vi "Main_RT_V2.vi"() -> ()   [LabVIEW 2018]
uses:
  enum_Main_RT_V2.ctl
  <vilib>/Platform/TimedLoop/XDataNode/timing_clust.ctl
  <vilib>/Platform/TimedLoop/XDataNode/nitl_modes.ctl
  <vilib>/Platform/TimedLoop/XDataNode/wakeup.ctl
  enum_bras.ctl
  <vilib>/myRIO/Instrument Drivers/Onboard IO/DIO/typedefs/DIO Reference.ctl
  <vilib>/myRIO/Common/Instrument Driver Framework/Utilities/typedefs/myRIO Generic Hardware Reference.ctl
  <vilib>/myRIO/Common/Instrument Driver Framework/Utilities/typedefs/Hardware Version Enum.ctl
  <vilib>/myRIO/Common/Instrument Driver Framework/Utilities/typedefs/myRIO v1.0 Reference.ctl
  <vilib>/myRIO/Common/Instrument Driver Framework/Utilities/typedefs/Generic FPGA Reference.ctl
  <vilib>/myRIO/Common/Instrument Driver Framework/myRIO v1.0/DIO/typedefs/DIO Channels List.ctl
  <vilib>/myRIO/Common/Instrument Driver Framework/myRIO v1.0/DIO/typedefs/DIO Channels Enum.ctl
  <vilib>/userdefined/High Color/nirio_resource_hc.ctl
  enum_RT_Virage.ctl
  enum_RT_Seaux.ctl
  enum_RT_recule.ctl
  enum_RT_trieur_Balles.ctl
  enum_RT_lanceur.ctl
  <vilib>/myRIO/Common/Instrument Driver Framework/Utilities/vis/Is FPGA Ref Available.vi
  <vilib>/myRIO/Common/Instrument Driver Framework/myRIO v1.0/DIO/vis/myRIO v1.1 Open DIO.vi
  <vilib>/myRIO/Instrument Drivers/Onboard IO/DIO/vis/Read.vi
  <vilib>/myRIO/Common/Instrument Driver Framework/Utilities/vis/Validate Channels.vi
  <vilib>/myRIO/Common/Instrument Driver Framework/myRIO v1.0/DIO/vis/myRIO v1.0 Reserve DIO.vi
  <vilib>/myRIO/Common/Instrument Driver Framework/myRIO v1.0/Resource Manager/vis/myRIO v1.0 Reserve Channel List.vi
  <vilib>/myRIO/Common/Instrument Driver Framework/myRIO v1.0/DIO/vis/myRIO v1.0 Build MUX Configuration DIO.vi
  <vilib>/myRIO/Common/Instrument Driver Framework/myRIO v1.0/Resource Manager/vis/myRIO v1.0 Reserve Channel.vi
  <vilib>/myRIO/Common/Instrument Driver Framework/myRIO v1.0/Resource Manager/vis/myRIO v1.0 Unreserve Channel.vi
  <vilib>/myRIO/Common/Instrument Driver Framework/myRIO v1.0/Resource Manager/vis/myRIO v1.0 Create Configuration List.vi
  <vilib>/myRIO/Common/Instrument Driver Framework/myRIO v1.0/Resource Manager/vis/myRIO v1.0 Build Mutex Name.vi
  <vilib>/Utility/VariantDataType/GetNumericInfo.vi
  <vilib>/Utility/error.llb/Error Cluster From Error Code.vi
  <vilib>/myRIO/Common/Instrument Driver Framework/myRIO v1.0/myRIO v1.1 Open.vi
  <vilib>/myRIO/Common/Instrument Driver Framework/Utilities/vis/IO Manager.vi
  <vilib>/myRIO/Common/Instrument Driver Framework/Utilities/vis/Configuration Manager.vi
  <vilib>/myRIO/Common/Instrument Driver Framework/myRIO v1.0/Resource Manager/vis/myRIO v1.0 Configure IO.vi
  <vilib>/myRIO/Common/Instrument Driver Framework/myRIO v1.0/myRIO v1.0 Close.vi
  <vilib>/myRIO/Common/Instrument Driver Framework/myRIO v1.0/DIO/vis/myRIO v1.0 Read DIO.vi
  <vilib>/Platform/TimedLoop/XDataNode/XDataNode.xnode
  <vilib>/myRIO/Express VI/Onboard Devices/Button/Button Express VI.xnode
  <vilib>/myRIO/Instrument Drivers/Onboard IO/DIO/vis/myRIO DIO Open.xnode
  <vilib>/Platform/TimedLoop/XDataNode/XDNodeRunTimeDep.lvlib
  <vilib>/myRIO/Instrument Drivers/Onboard IO/DIO/DIO.lvlib
panel:
  in  "stop":bool
  out "Sceaux":bool
  out "Lanceur de balles":bool
  out "Virage 4":bool
  out "Virage 3":bool
  out "Clapets 2":bool
  out "Trieur de Balles":bool
  out "Reculer":bool
  out "Virage 2":bool
  out "Virage 1":bool
  out "Clapets 1":bool
  out "Detection suiveur de ligne":bool[](array[boolean])
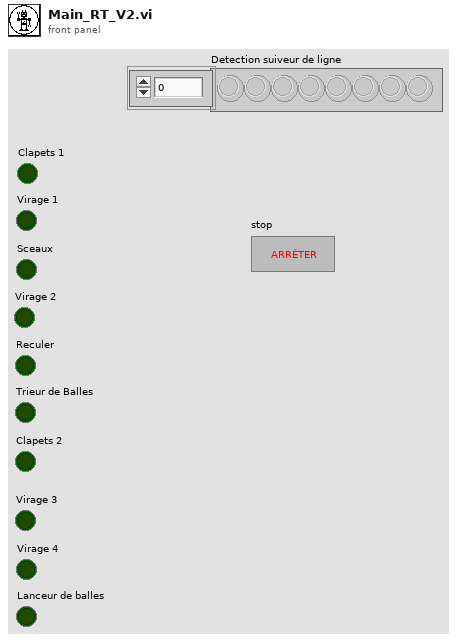
[diagram p1: front panel]
types:
  T1 = typedef "enum_Main_RT_V2.ctl" = enum16{"Initialisation", "Clapet 1", "Virage 1", "Seaux", "Virage 2", "Reculer", "Trieur Balles", "Avancer", "Clapet 2", "Virage 3", "Avancer 2", "Virage 4", "Lancer de Balles", "Arret du robot"}
  T2 = typedef "XDNodeRunTimeDep.lvlib/timing_clust.ctl" = cluster{"Expected End [f-1]":u64, "Actual End [f-1]":u64, "Finished Late? [f-1]":bool, "Expected End [i-1]":u64, "Actual End [i-1]":u64, "Finished Late? [i-1]":bool, "Expected Start [i]":u64, "Actual Start [i]":u64, "Expected Start [f]":u64, "Actual Start [f]":u64, "Source Name":string, "Structure Name":string, "Period":i64, "Deadline":i64, "Offset":i64, "Start":i64, "Priority":i32, "Timeout":i32, "Mode":T3, "Wakeup Reason":T4, "Error":errorcluster, "Source Type":string, "Secondary Source Type":string, "Global End Time":u64, "Global Start Time":u64, "Frame Duration":u64, "Iteration Duration":u64, "Assigned CPU":i32, "I/O Scan Engine Mode":u32}
  T3 = typedef "XDNodeRunTimeDep.lvlib/nitl_modes.ctl" = enum32{"No Change", "Process missed periods, maintain original phase", "Discard missed periods, maintain original phase", "Process missed periods, ignore original phase", "Discard missed periods, ignore original phase"}
  T4 = typedef "XDNodeRunTimeDep.lvlib/wakeup.ctl" = enum32{"Normal", "Aborted", "Asynchronous wakeup", "Timing source error", "Timed loop error", "Timeout"}
  T5 = typedef "enum_bras.ctl" = enum16{"Depart Bras", "Clapet Bras", "Inactif Bras", "Seaux Bras"}
  T6 = typedef "DIO.lvlib/DIO Reference.ctl" = cluster{"myRIO Reference":T7, "DIO Channels List":T11}
  T7 = typedef "myRIO Generic Hardware Reference.ctl" = cluster{"myRIO Model":T8, "myRIO Hardware Reference":T9}
  T8 = typedef "Hardware Version Enum.ctl" = enum16{"Unknown", "myRIO-1900", "myRIO-1950", "roboRIO", "NI ELVIS RIO CM", "ELVIS III"}
  T9 = typedef "myRIO v1.0 Reference.ctl" = cluster{"Generic FPGA Reference":T10, "Allow multiple opens":bool}
  T10 = typedef "Generic FPGA Reference.ctl" = refnum<k20>
  T11 = typedef "DIO Channels List.ctl" = T12[]
  T12 = typedef "DIO Channels Enum.ctl" = enum16{"Not Connected", "C/DIO0", "C/DIO1", "C/DIO2", "C/DIO3", "C/DIO4", "C/DIO5", "C/DIO6", "C/DIO7", "A/DIO0", "A/DIO1", "A/DIO2", "A/DIO3", "A/DIO4", "A/DIO5", "A/DIO6", "A/DIO7", "A/DIO8", "A/DIO9", "A/DIO10", "A/DIO11", "A/DIO12", "A/DIO13", "A/DIO14", "A/DIO15", "A/DIO16", "A/DIO17", "A/DIO18", "A/DIO19", "B/DIO0", "B/DIO1", "B/DIO2", "B/DIO3", "B/DIO4", "B/DIO5", "B/DIO6", "B/DIO7", "B/DIO8", "B/DIO9", "B/DIO10", "B/DIO11", "B/DIO12", "B/DIO13", "B/DIO14", "B/DIO15", "B/DIO16", "B/DIO17", "B/DIO18", "B/DIO19", "LED0", "LED1", "LED2", "LED3", "Button0", "DIO/DIO0", "DIO/DIO1", "DIO/DIO2", "DIO/DIO3", "DIO/DIO4", "DIO/DIO5", "DIO/DIO6", "DIO/DIO7", "DIO/DIO8", "DIO/DIO9", "SPI/CS0", "SPI/CS1", "SPI/CS2", "SPI/CS3", "LED RADIO (Green)", "LED RADIO (Red)", "LED COMM (Green)", "LED COMM (Red)", "LED MODE (Green)", "LED MODE (Red)"}
  T13 = typedef "nirio_resource_hc.ctl" = tag
  T14 = typedef "enum_RT_Virage.ctl" = enum16{"Avancer", "STOP", "Lacher Ligne", "Tourner"}
  T15 = typedef "enum_RT_Seaux.ctl" = enum16{"Avancé 1", "Ready to Start", "Stop moteur", "Bras Inactif 1", "Frappe sceau", "Bras Inactif 2", "Avancé 2"}
  T16 = typedef "enum_RT_recule.ctl" = enum16{"Avancer", "Reculer", "STOP"}
  T17 = typedef "enum_RT_trieur_Balles.ctl" = enum16{"Initialisation", "Couleur", "Rotation1", "Rotation2", "Ouverture", "Fermeture"}
  T18 = typedef "enum_RT_lanceur.ctl" = enum16{"eloignement", "arret_robot", "moteur_lanceur", "distributeur", "arret_distributeur_lanceur"}
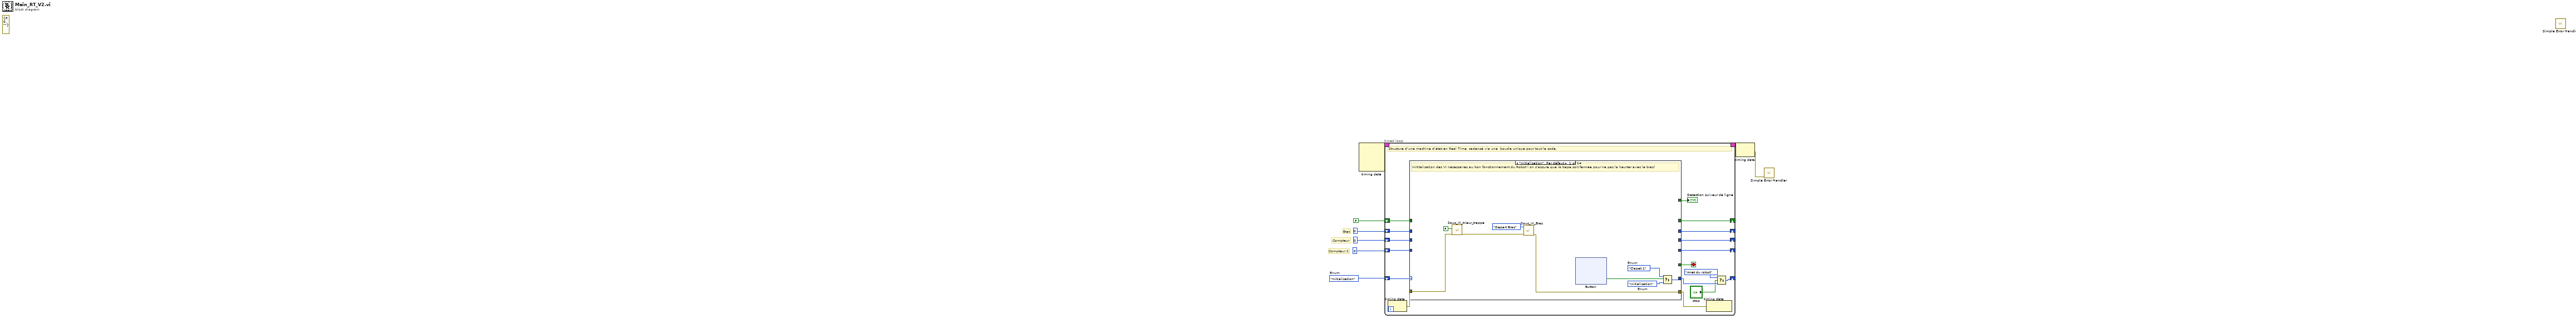
[diagram p0: block diagram]
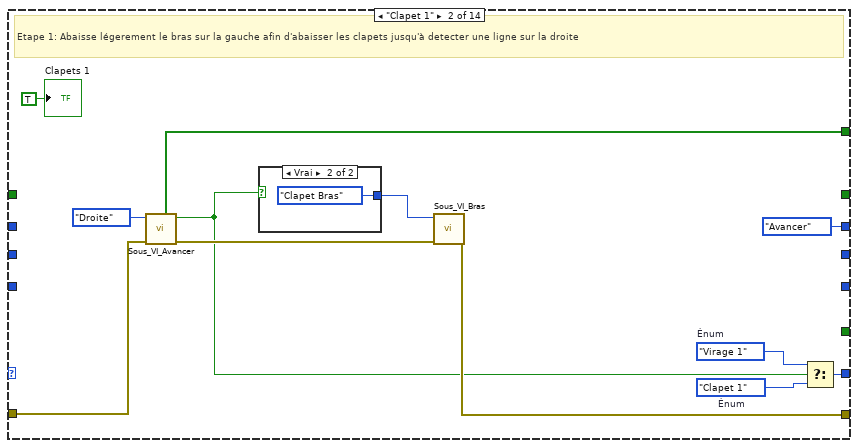
[diagram p2: hidden frame]
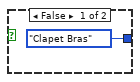
[diagram p3: hidden frame]
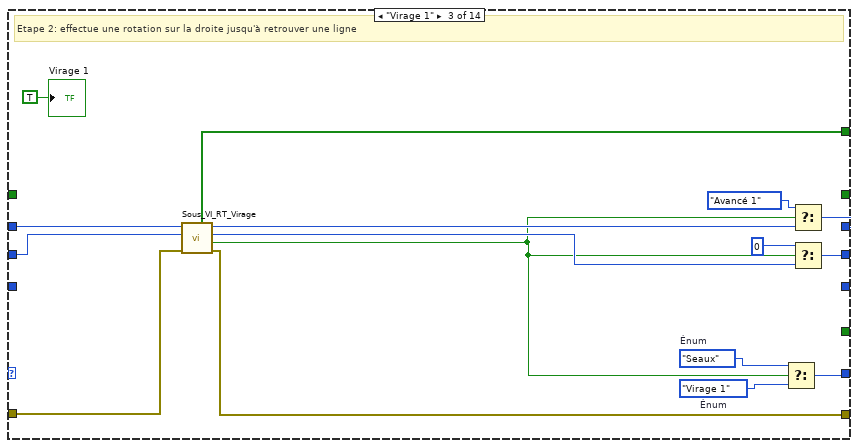
[diagram p4: hidden frame]
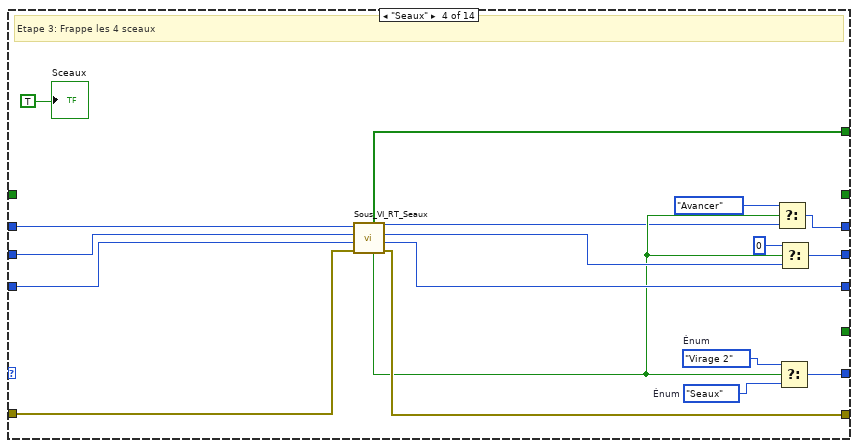
[diagram p5: hidden frame]
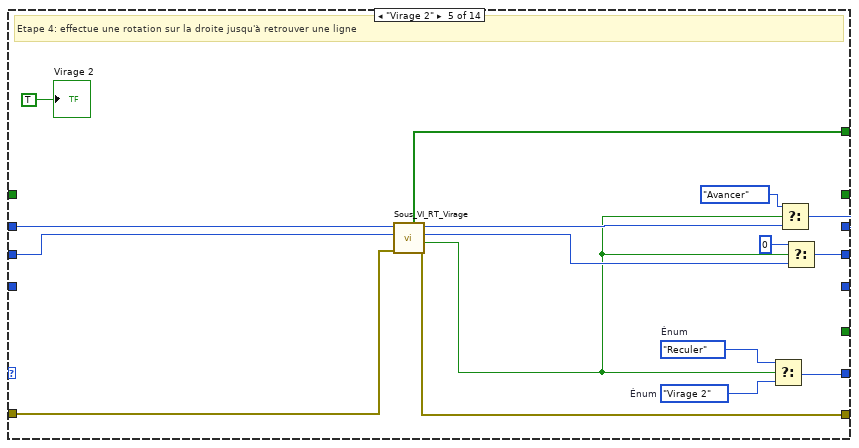
[diagram p6: hidden frame]
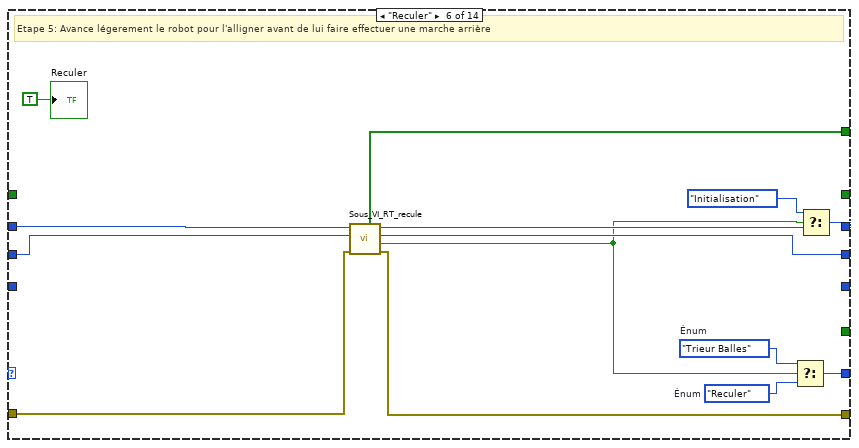
[diagram p7: hidden frame]
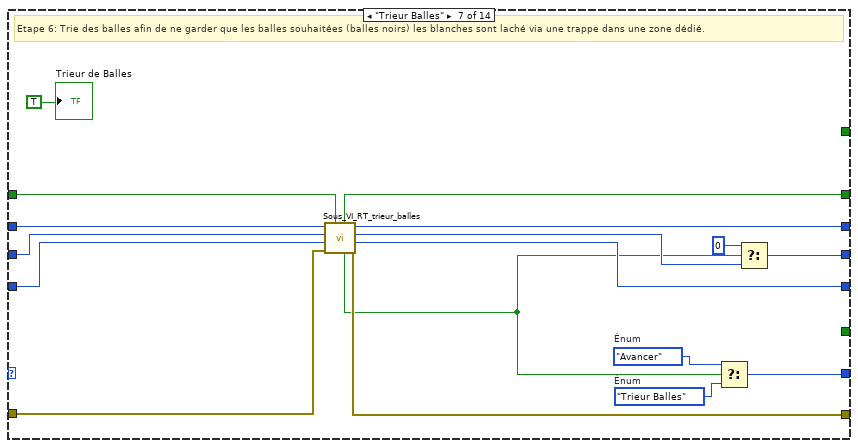
[diagram p8: hidden frame]
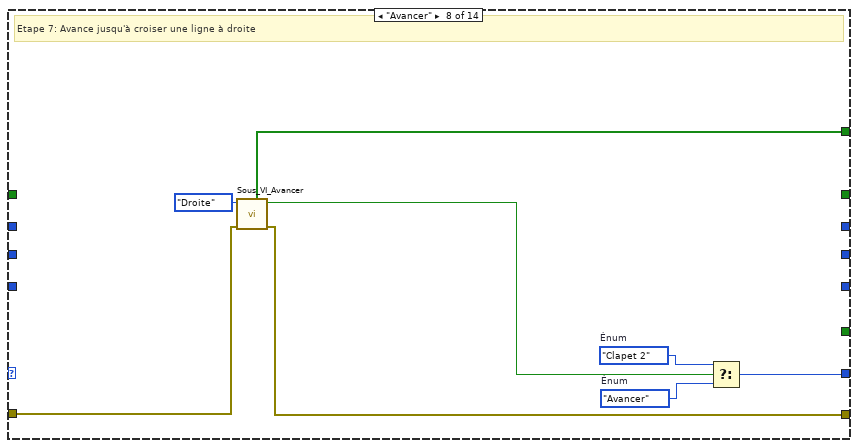
[diagram p9: hidden frame]
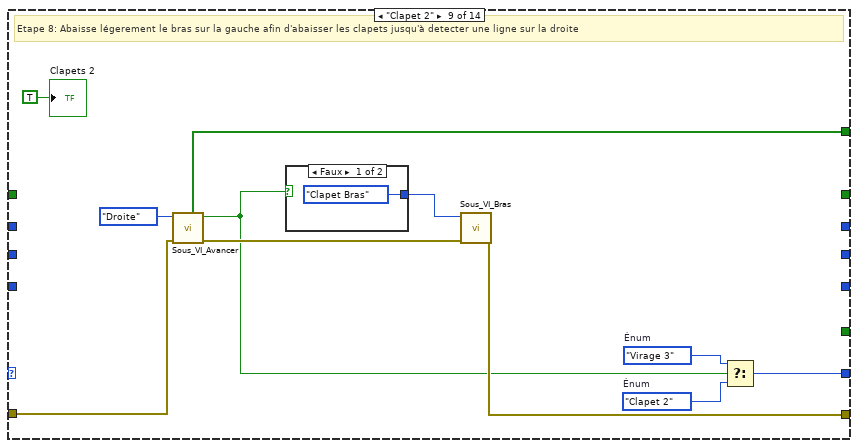
[diagram p10: hidden frame]
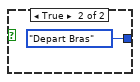
[diagram p11: hidden frame]
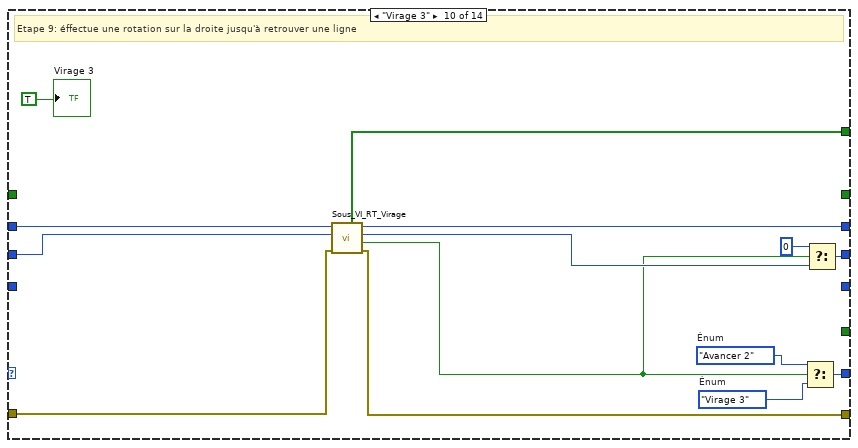
[diagram p12: hidden frame]
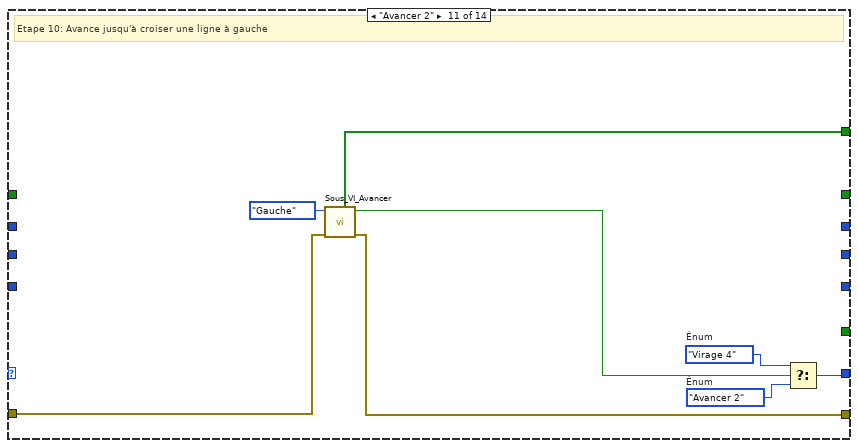
[diagram p13: hidden frame]
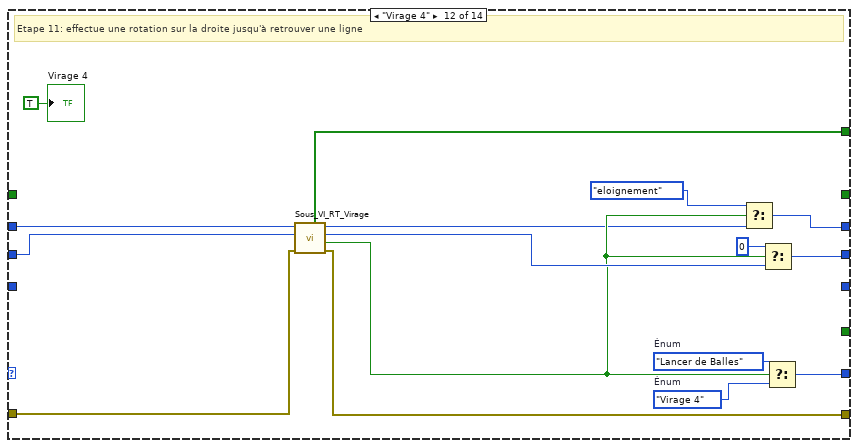
[diagram p14: hidden frame]
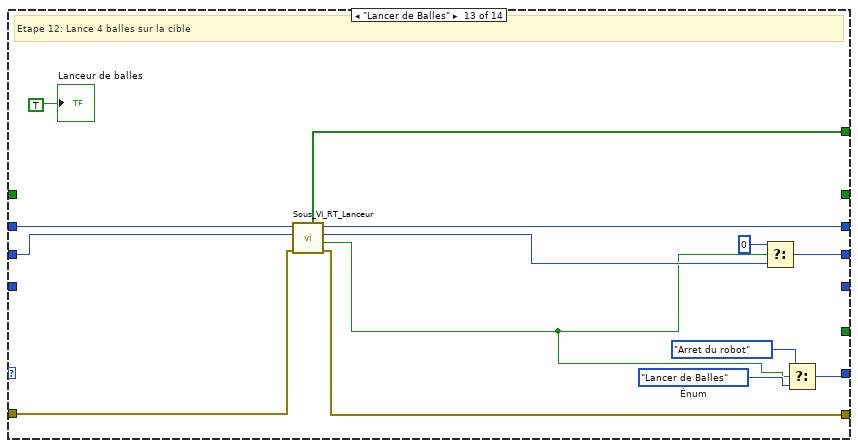
[diagram p15: hidden frame]
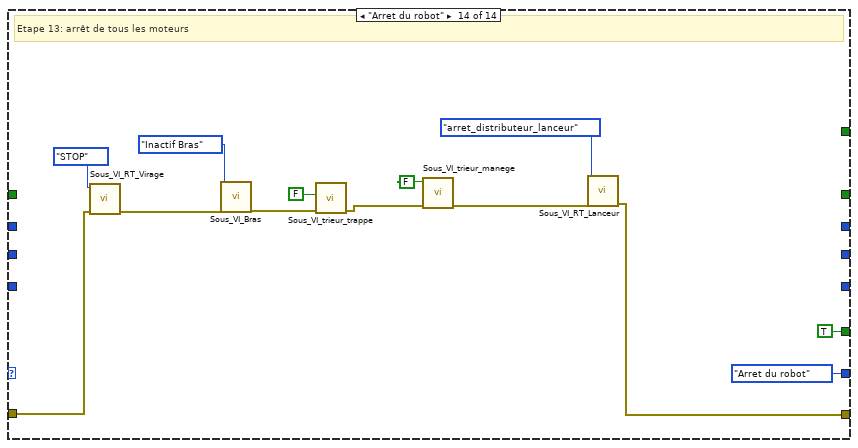
[diagram p16: hidden frame]
diagram:
  w1 = enum_Main_RT_V2."Initialisation"  # Énum
  (unwired) errorcluster {"status"=FALSE, "code"=0, "source"=""} ("error in (no error)")
  # "Compteur 2"
  # "Compteur"
  # "Etat"
  n1 = node-c288() -> (w8:T2)  [unwired: 4 in]
  n2 = timed-loop "Boucle cadencée" {
    timing: w8 -> [_]
    timing-out: [_] -> w7
    shift-right: [w22] -> _
    shift-left: u16 0 ("Etat OUT") -> [w20]
    shift-right: [w21] -> _
    shift-left: 0 -> [w19]
    shift-right: [w17] -> _
    shift-left: 0 -> [w18]
    shift-right: [w15] -> _
    shift-left: FALSE -> [w16]
    shift-right: [w12] -> _
    shift-left: w1 -> [w25]
    stop <- w14 stop-if-true
    # "Structure d'une machine d'état en Real Time, cadencé via une  boucle unique pour tout le code."
    n3 = node-c288() -> (w24:errorcluster)  [unwired: 1 in]
    n4 = case "Structure Condition" shown="\"Initialisation\", Par défaut" w25 {
      tunnel: w24 -> [w31 w78 w99 w117 w133 w144 w157 w171 w180 w196 w206 w221 w234 w250]
      tunnel: [w30 w77 w98 w116 w132 w143 w156 w170 w179 w195 w205 w220 w233 w240] -> w23
      tunnel: [_ enum_RT_Virage."Avancer" ("Etat IN") w90 w103 w121 w137 w163 _ _ w197 _ w211 w236 _] -> w22
      tunnel: [_ _ w96 w112 w128 w145 w154 _ _ w193 _ w218 w231 _] -> w21
      tunnel: w20 -> [_ _ w92 w108 w131 w147 w164 _ _ w199 _ w223 w237 _]
      tunnel: w19 -> [_ _ w97 w115 w130 w146 w162 _ _ w198 _ w222 w235 _]
      tunnel: w18 -> [_ _ _ w114 _ _ w161 _ _ _ _ _ _ _]
      tunnel: [_ _ _ w113 _ _ w160 _ _ _ _ _ _ _] -> w17
      tunnel: w16 -> [_ _ _ _ _ _ w159 _ _ _ _ _ _ _]
      tunnel: [_ _ _ _ _ _ w158 _ _ _ _ _ _ _] -> w15
      tunnel: [_ _ _ _ _ _ _ _ _ _ _ _ _ TRUE ("vi_fini")] -> w14
      tunnel: [w29 w73 w87 w107 w124 w141 w150 w169 w178 w189 w204 w215 w227 enum_Main_RT_V2."Arret du robot" ("Énum")] -> w11
      tunnel: [_ w75 w93 w109 w126 w142 _ w167 w176 w190 w202 w216 w229 _] -> w13
      frame "Initialisation", Default {
        w27 = enum_Main_RT_V2."Clapet 1"  # Énum
        w28 = enum_Main_RT_V2."Initialisation"  # Énum
        # "Inititalisation des VI nécessaires au bon fonctionnement du Robot ( on s'assure que la trape soit fermée pour ne pas la heurter avec le bras)"
        n5 = call "Sous_VI_trieur_trappe.vi"("error in (no error)"=w31, "Ouvrir"=FALSE) -> ("error out"=w32:errorcluster)  [unwired: 9 in]
        n6 = call "Sous_VI_Bras.vi"("error in (no error)"=w32, "Enum bras"=enum_bras."Depart Bras") -> ("error out"=w30:errorcluster)  [unwired: 9 in]
        n7 = xnode "Button"() -> ("Value"=w26:bool)  [unwired: 1 in, 1 out]
        n8 = Select(t=w27, s=w26, f=w28) -> (s? t:f=w29:T1)
      }
      frame "Clapet 1" {
        w71 = enum_Main_RT_V2."Clapet 1"  # Énum
        w70 = enum_Main_RT_V2."Virage 1"  # Énum
        # "Etape 1: Abaisse légerement le bras sur la gauche afin d'abaisser les clapets jusqu'à detecter une ligne sur la droite"
        n9 = call "Sous_VI_Avancer.vi"("error in (no error)"=w78, "Énum"=enum16{"Droite", "Gauche"}."Droite") -> ("error out"=w79:errorcluster, "Info de fin de Parcours"=w76:bool, "Détection ligne"=w75:bool[])  [unwired: 7 in]
        n10 = case shown="Vrai" w76 {
          tunnel: [enum_bras."Clapet Bras" ("Enum bras") enum_bras."Clapet Bras" ("Enum bras")] -> w80
          frame False {
          }
          frame True {
          }
        }
        n11 = call "Sous_VI_Bras.vi"("error in (no error)"=w79, "Enum bras"=w80) -> ("error out"=w77:errorcluster)  [unwired: 9 in]
        n12 = Select(t=w70, s=w76, f=w71) -> (s? t:f=w73:T1)
        "Clapets 1" <- TRUE
      }
      frame "Virage 1" {
        w85 = enum_Main_RT_V2."Virage 1"  # Énum
        w84 = enum_Main_RT_V2."Seaux"  # Énum
        # "Etape 2: effectue une rotation sur la droite jusqu'à retrouver une ligne"
        n13 = call "Sous_VI_RT_Virage.vi"("Erreur in"=w99, "Compteur IN"=w97, "Etat IN"=w92) -> ("Erreur out"=w98:errorcluster, "Information de fin de process"=w89:bool, "Compteur OUT"=w94:i32, "Etat OUT"=w91:T14, "Detection suiveur de ligne"=w93:bool[])  [unwired: 4 in]
        n14 = Select(t=w84, s=w89, f=w85) -> (s? t:f=w87:T1)
        n15 = Select(t=enum_RT_Seaux."Avancé 1" ("Etat IN"), s=w89, f=w91) -> (s? t:f=w90:u16)
        n16 = Select(t=0, s=w89, f=w94) -> (s? t:f=w96:i32)
        "Virage 1" <- TRUE
      }
      frame "Seaux" {
        w104 = enum_Main_RT_V2."Seaux"  # Énum
        w105 = enum_Main_RT_V2."Virage 2"  # Énum
        # "Etape 3: Frappe les 4 sceaux"
        n17 = call "Sous_VI_RT_Seaux.vi"("Erreur IN"=w117, "Nombre Sceau IN"=w114, "Compteur IN"=w115, "Etat IN"=w108) -> ("Erreur OUT"=w116:errorcluster, "Nombre Sceau OUT"=w113:i32, "Compteur OUT"=w110:i32, "Etat OUT"=w100:T15, "Indicateur de fin de process"=w102:bool, "Détection ligne"=w109:bool[])  [unwired: 2 in]
        n18 = Select(t=enum_RT_Virage."Avancer" ("Etat IN"), s=w102, f=w100) -> (s? t:f=w103:u16)
        n19 = Select(t=w105, s=w102, f=w104) -> (s? t:f=w107:T1)
        n20 = Select(t=0, s=w102, f=w110) -> (s? t:f=w112:i32)
        "Sceaux" <- TRUE
      }
      frame "Virage 2" {
        w122 = enum_Main_RT_V2."Reculer"  # Énum
        w123 = enum_Main_RT_V2."Virage 2"  # Énum
        # "Etape 4: effectue une rotation sur la droite jusqu'à retrouver une ligne"
        n21 = call "Sous_VI_RT_Virage.vi"("Erreur in"=w133, "Compteur IN"=w130, "Etat IN"=w131) -> ("Erreur out"=w132:errorcluster, "Information de fin de process"=w119:bool, "Compteur OUT"=w127:i32, "Etat OUT"=w120:T14, "Detection suiveur de ligne"=w126:bool[])  [unwired: 4 in]
        n22 = Select(t=w122, s=w119, f=w123) -> (s? t:f=w124:T1)
        n23 = Select(t=enum_RT_recule."Avancer", s=w119, f=w120) -> (s? t:f=w121:u16)
        n24 = Select(t=0, s=w119, f=w127) -> (s? t:f=w128:i32)
        "Virage 2" <- TRUE
      }
      frame "Reculer" {
        w139 = enum_Main_RT_V2."Reculer"  # Énum
        w138 = enum_Main_RT_V2."Trieur Balles"  # Énum
        # "Etape 5: Avance légerement le robot pour l'alligner avant de lui faire effectuer une marche arrière"
        n25 = call "Sous_VI_RT_recule.vi"("Erreur IN"=w144, "Compteur IN"=w146, "Etat IN"=w147) -> ("Erreur OUT"=w143:errorcluster, "Indicateur fin de process"=w134:bool, "Compteur OUT"=w145:i32, "Etat OUT"=w136:T16, "Detection suiveur de ligne"=w142:bool[])  [unwired: 4 in]
        n26 = Select(t=w138, s=w134, f=w139) -> (s? t:f=w141:T1)
        n27 = Select(t=enum_RT_trieur_Balles."Initialisation", s=w134, f=w136) -> (s? t:f=w137:u16)
        "Reculer" <- TRUE
      }
      frame "Trieur Balles" {
        w148 = enum_Main_RT_V2."Avancer"  # Énum
        w149 = enum_Main_RT_V2."Trieur Balles"  # Énum
        # "Etape 6: Trie des balles afin de ne garder que les balles souhaitées (balles noirs) les blanches sont laché via une trappe dans une zone dédié."
        n28 = call "Sous_VI_RT_trieur_balles.vi"("Détection couleur IN"=w159, "error in (no error)"=w157, "Nombre Balle IN"=w161, "Comteur IN"=w162, "Etat IN"=w164) -> ("error out"=w156:errorcluster, "Nombre Balle OUT"=w160:i32, "Comteur OUT"=w153:i32, "Etat OUT"=w163:T17, "Indicateur de fin de process"=w152:bool, "Détection couleur OUT"=w158:bool)  [unwired: 1 in]
        n29 = Select(t=w148, s=w152, f=w149) -> (s? t:f=w150:T1)
        n30 = Select(t=0, s=w152, f=w153) -> (s? t:f=w154:i32)
        "Trieur de Balles" <- TRUE
      }
      frame "Avancer" {
        w165 = enum_Main_RT_V2."Clapet 2"  # Énum
        w166 = enum_Main_RT_V2."Avancer"  # Énum
        # "Etape 7: Avance jusqu'à croiser une ligne à droite"
        n31 = call "Sous_VI_Avancer.vi"("error in (no error)"=w171, "Énum"=enum16{"Droite", "Gauche"}."Droite") -> ("error out"=w170:errorcluster, "Info de fin de Parcours"=w168:bool, "Détection ligne"=w167:bool[])  [unwired: 7 in]
        n32 = Select(t=w165, s=w168, f=w166) -> (s? t:f=w169:T1)
      }
      frame "Clapet 2" {
        w173 = enum_Main_RT_V2."Virage 3"  # Énum
        w174 = enum_Main_RT_V2."Clapet 2"  # Énum
        # "Etape 8: Abaisse légerement le bras sur la gauche afin d'abaisser les clapets jusqu'à detecter une ligne sur la droite"
        n33 = call "Sous_VI_Avancer.vi"("error in (no error)"=w180, "Énum"=enum16{"Droite", "Gauche"}."Droite") -> ("error out"=w181:errorcluster, "Info de fin de Parcours"=w177:bool, "Détection ligne"=w176:bool[])  [unwired: 7 in]
        n34 = case shown="Faux" w177 {
          tunnel: [enum_bras."Clapet Bras" ("Enum bras") enum_bras."Depart Bras" ("Enum bras")] -> w182
          frame False {
          }
          frame True {
          }
        }
        n35 = call "Sous_VI_Bras.vi"("error in (no error)"=w181, "Enum bras"=w182) -> ("error out"=w179:errorcluster)  [unwired: 9 in]
        n36 = Select(t=w173, s=w177, f=w174) -> (s? t:f=w178:T1)
        "Clapets 2" <- TRUE
      }
      frame "Virage 3" {
        w186 = enum_Main_RT_V2."Avancer 2"  # Énum
        w187 = enum_Main_RT_V2."Virage 3"  # Énum
        # "Etape 9: éffectue une rotation sur la droite jusqu'à retrouver une ligne"
        n37 = call "Sous_VI_RT_Virage.vi"("Erreur in"=w196, "Compteur IN"=w198, "Etat IN"=w199) -> ("Erreur out"=w195:errorcluster, "Information de fin de process"=w191:bool, "Compteur OUT"=w192:i32, "Etat OUT"=w197:T14, "Detection suiveur de ligne"=w190:bool[])  [unwired: 4 in]
        n38 = Select(t=w186, s=w191, f=w187) -> (s? t:f=w189:T1)
        n39 = Select(t=0, s=w191, f=w192) -> (s? t:f=w193:i32)
        "Virage 3" <- TRUE
      }
      frame "Avancer 2" {
        w200 = enum_Main_RT_V2."Virage 4"  # Énum
        w201 = enum_Main_RT_V2."Avancer 2"  # Énum
        # "Etape 10: Avance jusqu'à croiser une ligne à gauche"
        n40 = call "Sous_VI_Avancer.vi"("error in (no error)"=w206, "Énum"=enum16{"Droite", "Gauche"}."Gauche") -> ("error out"=w205:errorcluster, "Info de fin de Parcours"=w203:bool, "Détection ligne"=w202:bool[])  [unwired: 7 in]
        n41 = Select(t=w200, s=w203, f=w201) -> (s? t:f=w204:T1)
      }
      frame "Virage 4" {
        w213 = enum_Main_RT_V2."Lancer de Balles"  # Énum
        w212 = enum_Main_RT_V2."Virage 4"  # Énum
        # "Etape 11: effectue une rotation sur la droite jusqu'à retrouver une ligne"
        n42 = call "Sous_VI_RT_Virage.vi"("Erreur in"=w221, "Compteur IN"=w222, "Etat IN"=w223) -> ("Erreur out"=w220:errorcluster, "Information de fin de process"=w210:bool, "Compteur OUT"=w217:i32, "Etat OUT"=w208:T14, "Detection suiveur de ligne"=w216:bool[])  [unwired: 4 in]
        n43 = Select(t=enum_RT_lanceur."eloignement", s=w210, f=w208) -> (s? t:f=w211:u16)
        n44 = Select(t=0, s=w210, f=w217) -> (s? t:f=w218:i32)
        n45 = Select(t=w213, s=w210, f=w212) -> (s? t:f=w215:T1)
        "Virage 4" <- TRUE ("Virage 4")
      }
      frame "Lancer de Balles" {
        w226 = enum_Main_RT_V2."Lancer de Balles"  # Énum
        # "Etape 12: Lance 4 balles sur la cible"
        n46 = call "Sous_VI_RT_Lanceur.vi"("Erreur_in"=w234, "cpt_in"=w235, "enum_in"=w237) -> ("Erreur_out"=w233:errorcluster, "vi_fini"=w224:bool, "cpt_out"=w230:i32, "enum_out"=w236:T18, "Détection de ligne"=w229:bool[])  [unwired: 4 in]
        n47 = Select(t=0, s=w224, f=w230) -> (s? t:f=w231:i32)
        n48 = Select(t=enum_Main_RT_V2."Arret du robot" ("cas vrai"), s=w224, f=w226) -> (s? t:f=w227:T1)
        "Lanceur de balles" <- TRUE
      }
      frame "Arret du robot" {
        # "Etape 13: arrêt de tous les moteurs"
        n49 = call "Sous_VI_RT_Virage.vi"("Erreur in"=w250, "Etat IN"=enum_RT_Virage."STOP") -> ("Erreur out"=w249:errorcluster)  [unwired: 5 in, 4 out]
        n50 = call "Sous_VI_Bras.vi"("error in (no error)"=w249, "Enum bras"=enum_bras."Inactif Bras") -> ("error out"=w245:errorcluster)  [unwired: 9 in]
        n51 = call "Sous_VI_trieur_trappe.vi"("error in (no error)"=w245, "Ouvrir"=FALSE) -> ("error out"=w243:errorcluster)  [unwired: 9 in]
        n52 = call "Sous_VI_trieur_manege.vi"("error in (no error)"=w243, "ON/OFF"=FALSE) -> ("error out"=w242:errorcluster)  [unwired: 9 in]
        n53 = call "Sous_VI_RT_Lanceur.vi"("Erreur_in"=w242, "enum_in"=enum_RT_lanceur."arret_distributeur_lanceur") -> ("Erreur_out"=w240:errorcluster)  [unwired: 5 in, 4 out]
      }
    }
    "Detection suiveur de ligne" <- w13
    n54 = node-c288(w23) -> ()  [unwired: 1 out]
    n55 = Select(t=enum_Main_RT_V2."Arret du robot" ("cas vrai"), s="stop", f=w11) -> (s? t:f=w12:T1)
  }
  n56 = node-c288(w7) -> (w3:errorcluster)
  n57 = call <vilib>:"Simple Error Handler.vi"("error in (no error)"=w3) -> ()  [unwired: 4 in, 5 out]
  n58 = call <vilib>:"Simple Error Handler.vi"() -> ()  [unwired: 5 in, 5 out]
